vi "Own20261012_GetPropertyItemInfo.vi"() -> ()   [LabVIEW 2024]
uses:
  <vilib>/_script/All Supported PropertiesOrMethods TypeDefs/ASPM_UniqueIDStringDatanameShortnameLongname.ctl
panel:
  out "error out":errorcluster caption="错误输出"
  out "property":T1 caption="属性"
  out "is_write":bool
  in  "property_item_id":u32
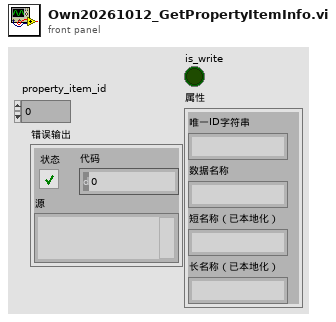
[diagram p1: front panel]
types:
  T1 = typedef "ASPM_UniqueIDStringDatanameShortnameLongname.ctl" = cluster{"Unique ID string":string, "Data name":string, "Short name (localized)":string, "Long name (localized)":string}
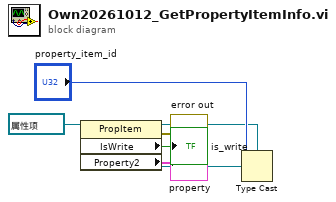
[diagram p0: block diagram]
diagram:
  n1 = Type Cast(type=refnum<vi> refnum ("引用"), x="property_item_id") -> (*(type *) &x=w4:refnum<vi>)
  n2 = property class="PropItem"(reference=w4) -> (error out=→"error out":errorcluster, "IsWrite"=→"is_write":bool, "Property2"=→"property":T1)  [unwired: 1 in, 1 out]
